vi "VHist - Interpolate multi DBL History.vi"(6 "method (linear)":T1(ring), 8 "error in":errorcluster, 9 "time stamp (0: now)":dbl format="%<%H:%M:%S%2u\n%d/%m/%Y>T", 10 "multiple history data":cluster{"history data":dbl[]}[](array[cluster]) {"history data" format="%.2f"}, 11 "time stamps":dbl[](array[numeric]) format="%<%H:%M:%S%2u\n%d/%m/%Y>T") -> (0 "error out":errorcluster, 2 "multiple history data out":cluster{"history data":dbl[]}[](array[cluster]) {"history data" format="%.2f"}, 3 "time stamps out":dbl[](array[numeric]) format="%<%H:%M:%S%2u\n%d/%m/%Y>T")   [LabVIEW 2021]
doc: "The VI inserts the specified timestamp and either interpolated or extrapolated values at this timestamp into an appropriate position in multiple DBL history. Interpolation method can be linear (by default), spline, polynominal or rational.\n\n::: CalcExpress Toolkit :::\nCopyright (c) 2000-2026 Konstantin Shifershteyn. All rights reserved."
uses:
  <vilib>/Analysis/NI_AALPro.lvlib
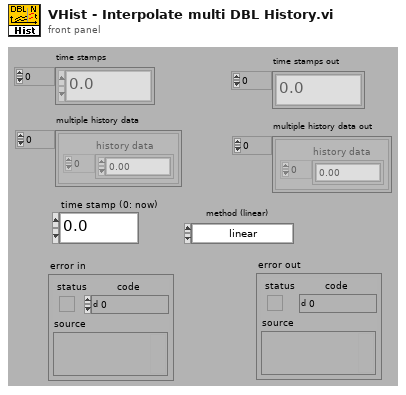
[diagram p1: front panel]
types:
  T1 = enum16{"linear", "spline", "polynominal", "rational"}
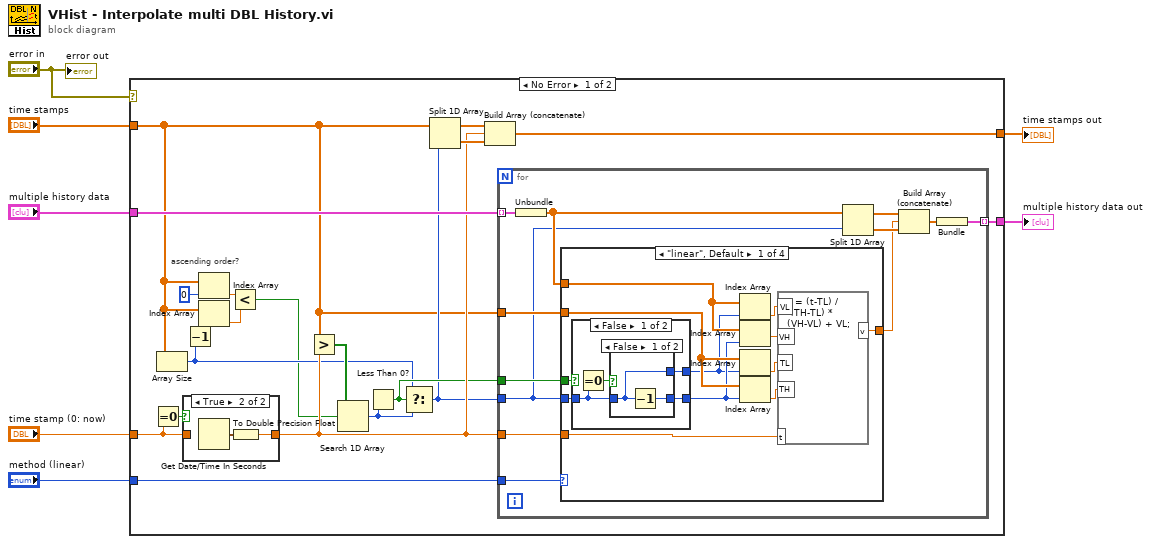
[diagram p0: block diagram]
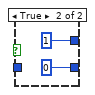
[diagram p2: hidden frame]
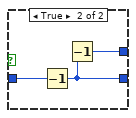
[diagram p3: hidden frame]
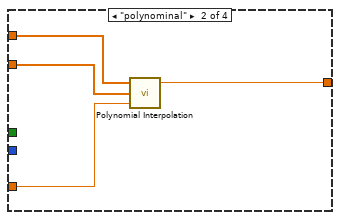
[diagram p4: hidden frame]
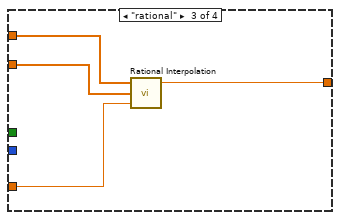
[diagram p5: hidden frame]
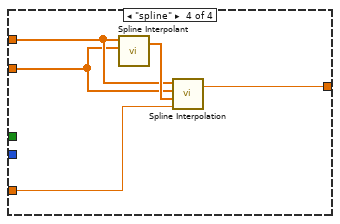
[diagram p6: hidden frame]
diagram:
  n1 = case shown="No Error" "error in" {
    tunnel: "multiple history data" -> [w26 w80]
    tunnel: [w23 w79] -> w7
    tunnel: [w22 w80] -> w3
    tunnel: "time stamps" -> [w9 w79]
    tunnel: "time stamp (0: now)" -> [w17 _]
    tunnel: "method (linear)" -> [w8 _]
    frame No Error {
      # "ascending order?"
      n2 = Equal To 0?(x=w17) -> (x = 0?=w27:bool)
      n3 = Array Size(array=w9) -> (size(s)=w11:i32)
      n4 = case shown="True" w27 {
        tunnel: [w76 w78] -> w20
        tunnel: w17 -> [w76 _]
        frame False {
        }
        frame True {
          n5 = Get Date/Time In Seconds() -> (seconds since 1Jan1904=w77:timestamp)
          n6 = To Double Precision Float(number=w77) -> (double precision float=w78:dbl)
        }
      }
      n7 = Decrement(x=w11) -> (x-1=w12:i32)
      n8 = Index Array(array=w9, index=0) -> (element=w14:dbl)
      n9 = Index Array(array=w9, index=w12) -> (element=w13:dbl)
      n10 = Less?(x=w14, y=w13) -> (x < y?=w10:bool)
      n11 = Greater?(x=w9, y=w20) -> (0:w21:bool[])
      n12 = Search 1D Array(1D array=w21, element=w10) -> (index of element=w19:i32)  [unwired: 1 in]
      n13 = Less Than 0?(x=w19) -> (x < 0?=w18:bool)
      n14 = Select(t=w11, s=w18, f=w19) -> (s? t:f=w16:i32)
      n15 = Split 1D Array(array=w9, index=w16) -> (first subarray=w25:dbl[], second subarray=w24:dbl[])
      n16 = Build Array (concatenate)(w25, w20, w24) -> (w23:dbl[])
      n17 = for {
        tunnel: w8 -> [w39]
        tunnel: w26 -> [w38] mode=indexing
        tunnel: [w29] -> w22 mode=indexing
        tunnel: w20 -> [w33]
        tunnel: w9 -> [w32]
        tunnel: w18 -> [w31]
        tunnel: w16 -> [w28]
        n18 = Unbundle(w38) -> ("history data"=w30:dbl[])
        n19 = case shown="\"linear\", Default" w39 {
          tunnel: w32 -> [w49 w66 w69 w72]
          tunnel: w33 -> [w51 w65 w68 w74]
          tunnel: w30 -> [w44 w64 w70 w73]
          tunnel: [w50 w63 w67 w71] -> w34
          tunnel: w31 -> [w43 _ _ _]
          tunnel: w28 -> [w42 _ _ _]
          frame "linear", Default {
            n20 = case shown="False" w43 {
              tunnel: w42 -> [w52 w62]
              tunnel: [w55 w61] -> w41
              tunnel: [w54 w60] -> w40
              frame False {
                n21 = Equal To 0?(x=w52) -> (x = 0?=w53:bool)
                n22 = case shown="False" w53 {
                  tunnel: [w56 0] -> w55
                  tunnel: [w57 1] -> w54
                  tunnel: w52 -> [w57 _]
                  frame False {
                    n23 = Decrement(x=w57) -> (x-1=w56:i32)
                  }
                  frame True {
                  }
                }
              }
              frame True {
                n24 = Decrement(x=w62) -> (x-1=w61:i32)
                n25 = Decrement(x=w61) -> (x-1=w60:i32)
              }
            }
            n26 = Index Array(array=w44, index=w40) -> (element=w48:dbl)
            n27 = Index Array(array=w44, index=w41) -> (element=w47:dbl)
            n28 = Index Array(array=w49, index=w40) -> (element=w46:dbl)
            n29 = Index Array(array=w49, index=w41) -> (element=w45:dbl)
            n30 = formula code="v = (t-TL) /\n (TH-TL) * \n(VH-VL) + VL;"("TH"=w45, "TL"=w46, "VH"=w47, "VL"=w48, "t"=w51) -> ("v"=w50:dbl)
          }
          frame "polynominal" {
            n31 = call <vilib>:"Polynomial Interpolation.vi"("x value"=w65, "X"=w66, "Y"=w64) -> ("interpolation value"=w63:dbl)  [unwired: 2 out]
          }
          frame "rational" {
            n32 = call <vilib>:"Rational Interpolation.vi"("x value"=w68, "X"=w69, "Y"=w70) -> ("interpolation value"=w67:dbl)  [unwired: 2 out]
          }
          frame "spline" {
            n33 = call <vilib>:"Spline Interpolant.vi"("X"=w72, "Y"=w73) -> ("Interpolant"=w75:dbl[])  [unwired: 2 in, 1 out]
            n34 = call <vilib>:"Spline Interpolation.vi"("x value"=w74, "Interpolant"=w75, "X"=w72, "Y"=w73) -> ("interpolation value"=w71:dbl)  [unwired: 1 out]
          }
        }
        n35 = Split 1D Array(array=w30, index=w28) -> (first subarray=w37:dbl[], second subarray=w36:dbl[])
        n36 = Build Array (concatenate)(w37, w34, w36) -> (w35:dbl[])
        n37 = Bundle(w35) -> (w29:cluster{dbl[]})  [unwired: 1 in]
      }
    }
    frame Error {
    }
  }
  "time stamps out" <- w7
  "multiple history data out" <- w3
  "error out" <- "error in"
